vi "track_chunk.read.vi"(8 "error in":errorcluster, 10 "midi-file-events in":refnum<class "midi-file-events.lvclass">, 11 "midi-file in":refnum<class "midi-file.lvclass">) -> (0 "error out":errorcluster, 2 "midi-file-events out":refnum<class "midi-file-events.lvclass">, 3 "midi-file out":refnum<class "midi-file.lvclass">)   [LabVIEW 2020, in "midi-file.lvclass"]
uses:
  midi-file.lvclass
  midi-file-events/midi-file-events.lvclass
  midi-file.lvclass/midi-file.ctl
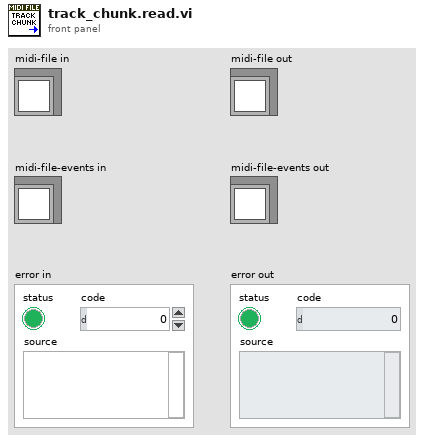
[diagram p1: front panel]
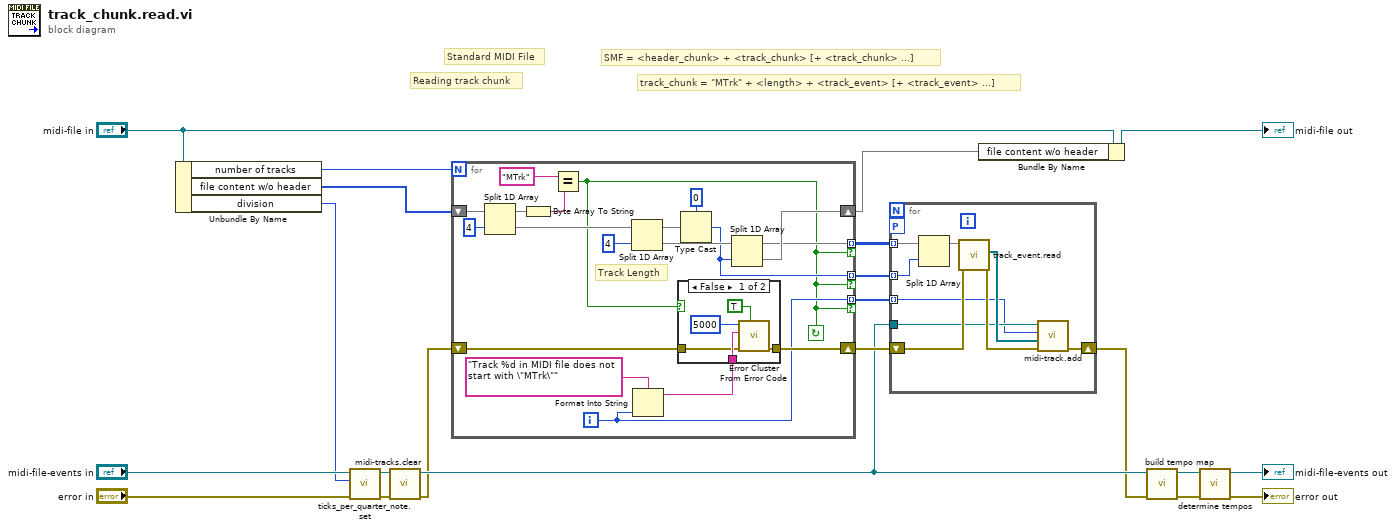
[diagram p0: block diagram]
diagram:
  # "track_chunk = \"MTrk\" + <length> + <track_event> [+ <track_event> ...]"
  # "Reading track chunk"
  # "Standard MIDI File"
  # "SMF = <header_chunk> + <track_chunk> [+ <track_chunk> ...]"
  n1 = Unbundle By Name("midi-file in") -> ("number of tracks"=w16:i16, "file content w/o header"=w19:u8[], "division"=w10:i16)
  n2 = call "ticks_per_quarter_note.set.vi"("error in (no error)"="error in", "ticks per quarter note (division)"=w10, "midi-file-events in"="midi-file-events in") -> ("error out"=w4:errorcluster, "midi-file-events out"=w12:refnum<class "midi-file-events.lvclass">)  [unwired: 7 in]
  n3 = call "midi-tracks.clear.vi"("error in (no error)"=w4, "midi-file-events in"=w12) -> ("error out"=w2:errorcluster, "midi-file-events out"=w8:refnum<class "midi-file-events.lvclass">)  [unwired: 8 in]
  n4 = for {
    N: w16 -> [_]
    shift-right: [w32] -> w15
    shift-left: w19 -> [w35]
    tunnel: [w31] -> w18 mode=indexing if=w22
    tunnel: [w30] -> w17 mode=indexing if=w22
    shift-right: [w25] -> w14
    shift-left: w2 -> [w24]
    tunnel: [w23] -> w13 mode=indexing if=w22
    i -> [w23]
    stop <- w22 continue-if-true
    # "Track Length"
    n5 = Split 1D Array(array=w35, index=4) -> (first subarray=w34:u8[], second subarray=w33:u8[])
    n6 = Byte Array To String(unsigned byte array=w34) -> (string=w29:string)
    n7 = Equal?(x="MTrk", y=w29) -> (x = y?=w22:bool)
    n8 = Split 1D Array(array=w33, index=4) -> (first subarray=w38:u8[], second subarray=w40:u8[])
    n9 = Format Into String(format string="Track %d in MIDI file does not start with \"MTrk\"" ("error message (\"\")"), w23) -> (resulting string=w26:string)  [unwired: 2 in, 1 out]
    n10 = case shown="False" w22 {
      tunnel: w26 -> [w44 _]
      tunnel: [w43 w46] -> w25
      tunnel: w24 -> [w42 w46]
      frame False {
        n11 = call <vilib>:"Error Cluster From Error Code.vi"("show call chain? (False)"=TRUE, "error in (no error)"=w42, "error message (\"\")"=w44, "error code (0)"=5000) -> ("error out"=w43:errorcluster)  [unwired: 5 in]
      }
      frame True {
      }
    }
    n12 = Type Cast(type=0, x=w38) -> (*(type *) &x=w30:i32)
    n13 = Split 1D Array(array=w40, index=w30) -> (first subarray=w31:u8[], second subarray=w32:u8[])
  }
  n14 = for {
    workers-P: _ -> [_]
    tunnel: w18 -> [w54] mode=indexing
    tunnel: w17 -> [w53] mode=indexing
    shift-right: [w49] -> w6
    shift-left: w14 -> [w52]
    tunnel: w8 -> [w48]
    tunnel: w13 -> [w47] mode=indexing
    n15 = Split 1D Array(array=w54, index=w53) -> (first subarray=w55:u8[])  [unwired: 1 out]
    n16 = call "track_event.read.vi"("error in"=w52, "Track Chunk Core"=w55) -> ("error out"=w50:errorcluster, "file events"=w51:refnum<class "midi-file-event.lvclass">[])  [unwired: 7 in, 1 out]
    n17 = call "midi-track.add.vi"("error in (no error)"=w50, "Track Events"=w51, "Track Number"=w47, "midi-file-events in"=w48) -> ("error out"=w49:errorcluster)  [unwired: 6 in, 1 out]
  }
  n18 = Bundle By Name(cluster="midi-file in", "file content w/o header"=w15) -> (→"midi-file out":refnum<class "midi-file.lvclass">)
  n19 = call "build tempo map.vi"("error in (no error)"=w6, "midi-file-events in"=w8) -> ("error out"=w5:errorcluster, "midi-file-events out"=w7:refnum<class "midi-file-events.lvclass">)  [unwired: 8 in]
  n20 = call "determine tempos.vi"("error in (no error)"=w5, "midi-file-events in"=w7) -> ("error out"=→"error out":errorcluster, "midi-file-events out"=→"midi-file-events out":refnum<class "midi-file-events.lvclass">)  [unwired: 7 in, 1 out]
